vi "Main Page.vi"(8 "error in (no error)":errorcluster, 11 "Node Ptr":T4 format="%.0x") -> (0 "error out":errorcluster)   [LabVIEW 2024, in "Diagnostics Addon System Explorer.lvlib"]
uses:
  Diagnostics Addon System Explorer.lvlib
  <vilib>/NI VeriStand/Custom Device API/Custom Device API.lvlib
  Types/FG.Action.ctl
  Addon Shared/Types/986x.ctl
  Addon Shared/Diagnostics Addon Shared.lvlib
  <vilib>/NI/NI VeriStand Hardware Resource Discovery/NIVS Hardware Discovery.lvlib
  <vilib>/NI/NI VeriStand Hardware Resource Discovery/_Types/Filter Type.ctl
  Addon Shared/SubVIs/Constants.vi
  <vilib>/NI VeriStand/Custom Device API/Custom Device Item Ref.ctl
  Addon Shared/Types/Protocol.ctl
  Addon Shared/Types/Transport.ctl
panel:
  in  "Tab Control":T1(tab)
  in  "Dynamic Port":bool=TRUE
  in  "DoIP Version":u16(ring)=2 items=["2010"=1, "2012"=2]
  in  "Address":string
  in  "FD ISO Mode":u32(ring) items=["ISO", "Non ISO", "ISO Legacy"]
  in  "CAN Browse":bool
  out "Version":string
  in  "Termination":enum16{"Off", "On"}(ring)
  in  "Name":string
  in  "Description":string
  out "Diagnostic Protocol":T2
  in  "Port":string
  in  "Baud Rate":u64=250000
  in  "Enable Stream":bool
  in  "FD Baud Rate":u64=250000
  in  "Max DLC":u16
  in  "IO Mode":u32(ring) items=["CAN 2.0", "CAN FD", "CAN FD+BRS"]
  in  "Transport Protocol":T3
  in  "Source Address":u16=3584 format="%.0x"
  in  "Timeout":u32 caption="Comm Timeout (ms)"
  in  "Fill Byte":u8=255 format="%.0x"
  in  "Fill Frame":bool
  in  "VW TP Channel ID":u32 format="%.0x"
  in  "Receive UUDT ID":u32 format="%.0x"
  in  "Receive Extension":u8 format="%.0x"
  in  "Receive ID":u32 format="%.0x"
  in  "Transmit Extension":u8 format="%.0x"
  in  "Transmit ID":u32 format="%.0x"
  in  "NAD":u8
  in  "LIN Cluster":refnum<k21>
  in  "RIO Browse":bool
  in  "RIO Device":string
  in  "Enable Bitfile":bool
  in  "Bitfile Path":path
  in  "Header":cluster{"Section Name":string}={"Section Name"="Addon Settings"}
  in  "SHDocVw.IWebBrowser":refnum<k7>(container)
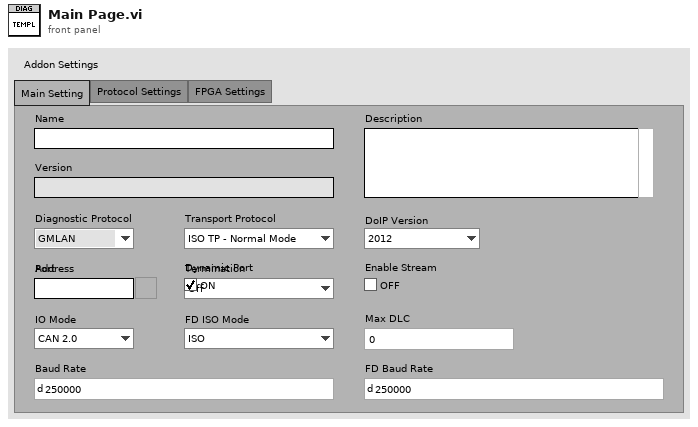
[diagram p1: front panel]
types:
  T1 = enum32{"Main Setting", "Protocol Settings", "FPGA Settings"}
  T2 = typedef "Diagnostics Addon Shared.lvlib/Protocol.ctl" = enum16{"GMLAN", "KWP-2000", "UDS", "User-Defined"}
  T3 = typedef "Diagnostics Addon Shared.lvlib/Transport.ctl" = enum16{"ISO TP - Normal Mode", "ISO TP - Mixed Mode", "VW TP 2.0", "Diagnostics on IP", "ISO TP LIN"}
  T4 = typedef "Custom Device API.lvlib/Custom Device Item Ref.ctl" = u64
  T5 = typedef "Diagnostics Addon System Explorer.lvlib/FG.Action.ctl" = enum16{"Get", "Set"}
  T6 = typedef "Custom Device API.lvlib/Custom Device Item Info.ctl" = cluster{"Name":string, "Is Channel":bool, "GUID":string, "Is Waveform":bool}
  T7 = typedef "Diagnostics Addon Shared.lvlib/986x.ctl" = cluster{"Enable":bool, "RIO Device":string, "Bitfile":path}
  T8 = typedef "Diagnostics Addon Shared.lvlib/CAN.ctl" = cluster{"Interface":T9, "Baud Rate":u64, "Diagnostic Protocol":T2, "Transport Protocol":T3, "Transmit ID":u32, "Receive ID":u32, "Transmit Extension":u8, "Receive Extension":u8, "Receive UUDT ID":u32, "Enable Stream":bool, "VW TP Channel ID":u32, "Fill Frame":bool, "Fill Byte":u8, "Termination":bool, "LIN Cluster":refnum<k21>, "NAD":u8, "IO Mode":u32, "Max DLC":u16, "FD Baud Rate":u64, "Timeout":u32, "FD ISO Mode":u32, "DoIP Address":string, "DoIP Source Address":u16, "DoIP Dynamic Port":bool, "DoIP Version":u16}
  T9 = typedef "Diagnostics Addon Shared.lvlib/CAN.Interface.ctl" = string
  T10 = typedef "NIVS Hardware Discovery.lvlib/Filter Type.ctl" = enum16{"Device Category", "Product Name", "Ethernet", "XNET", "VISA", "FPGA", "EtherCAT Master", "DAQmx", "GPIB", "Serial"}
  T11 = typedef "Custom Device API.lvlib/Custom Device Commands.ctl" = enum16{"Default", "Item renamed", "Shutdown", "Dynamic button pressed"}
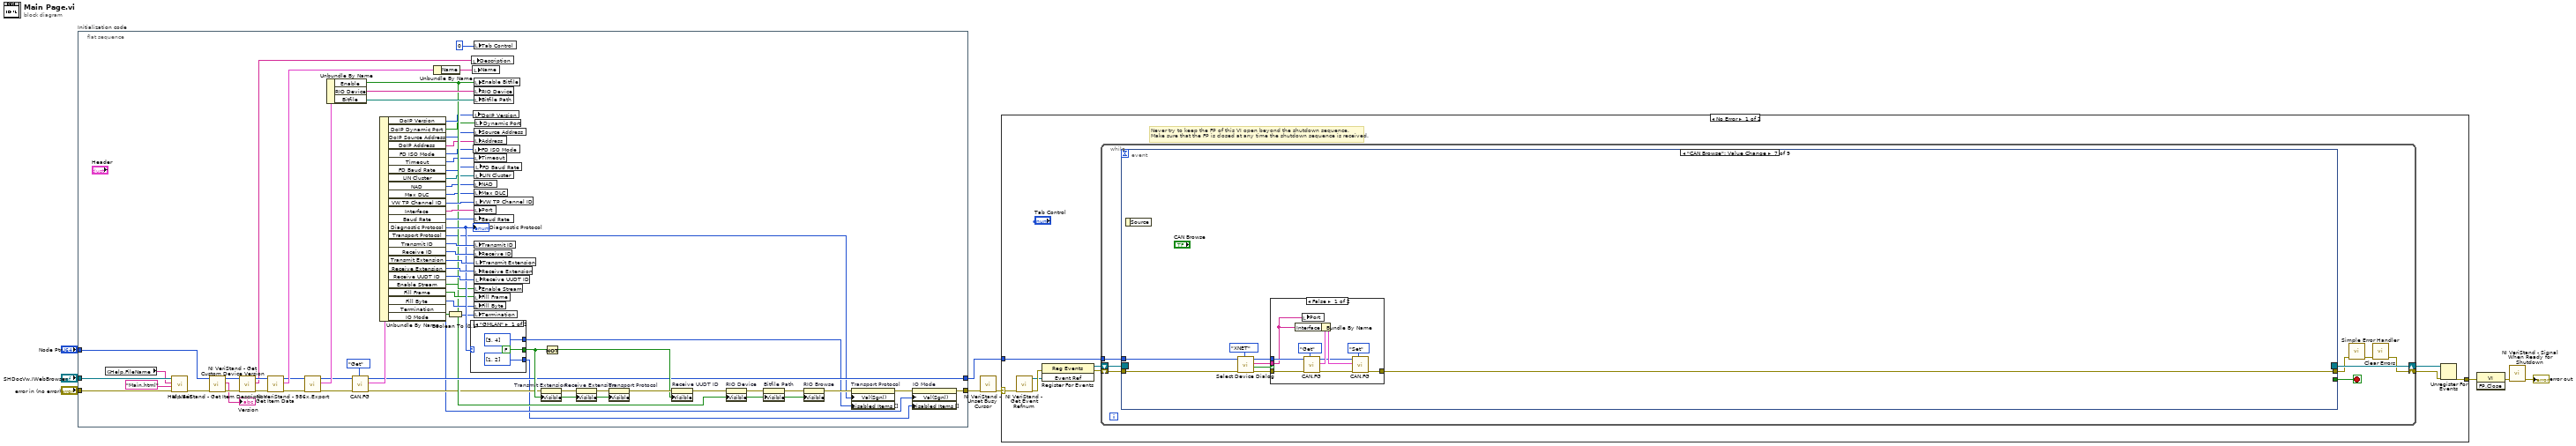
[diagram p0: block diagram]
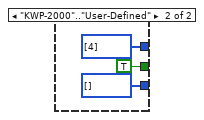
[diagram p2: hidden frame]
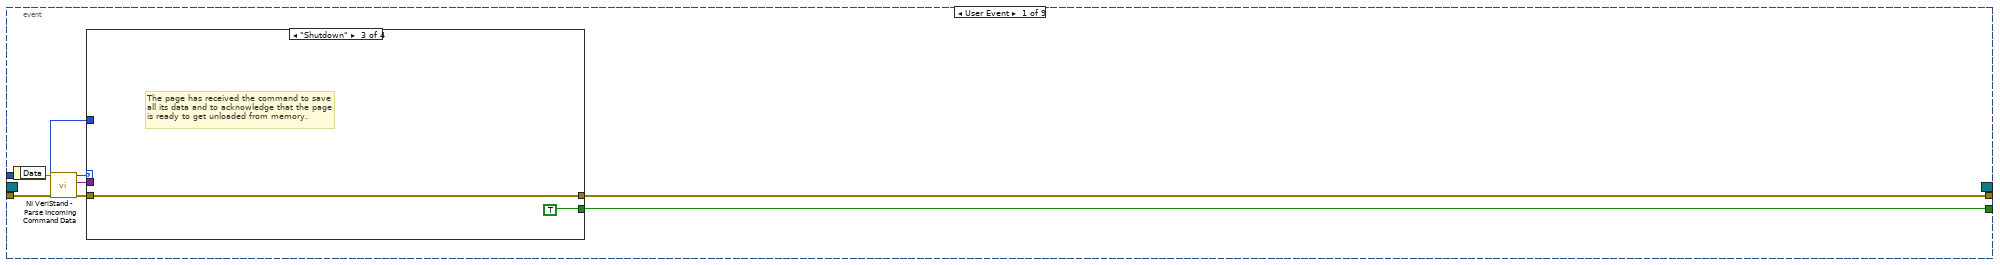
[diagram p3: hidden frame]
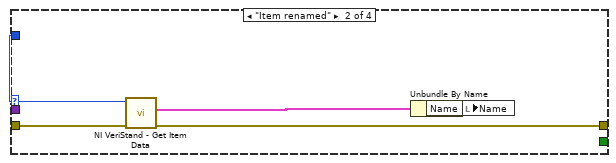
[diagram p5: hidden frame]
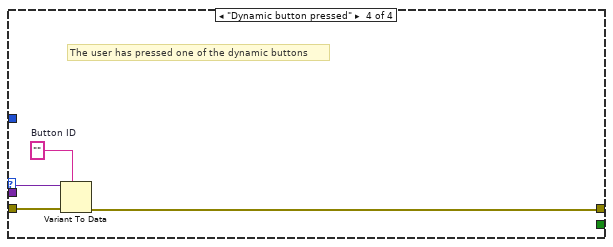
[diagram p6: hidden frame]
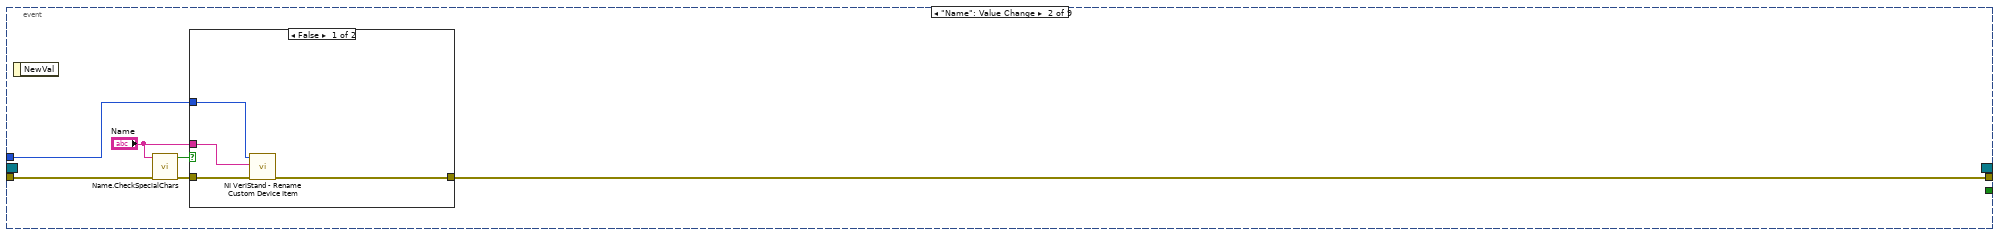
[diagram p7: hidden frame]
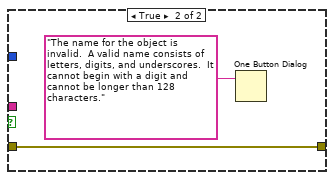
[diagram p8: hidden frame]
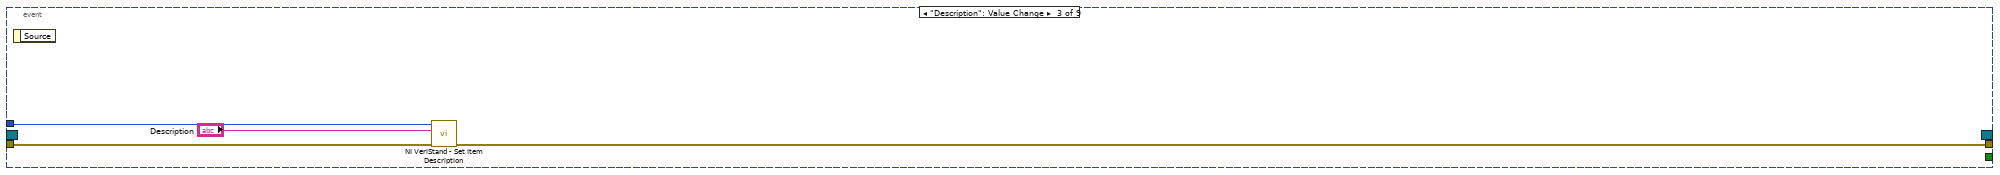
[diagram p9: hidden frame]
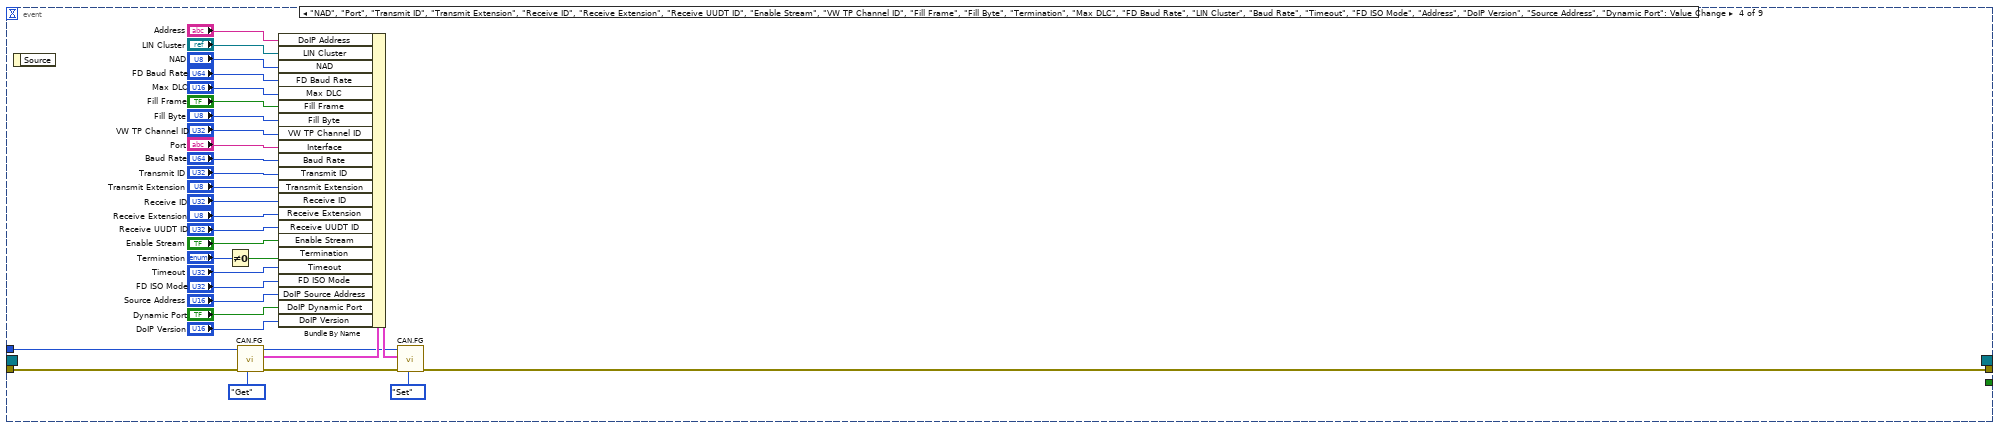
[diagram p10: hidden frame]
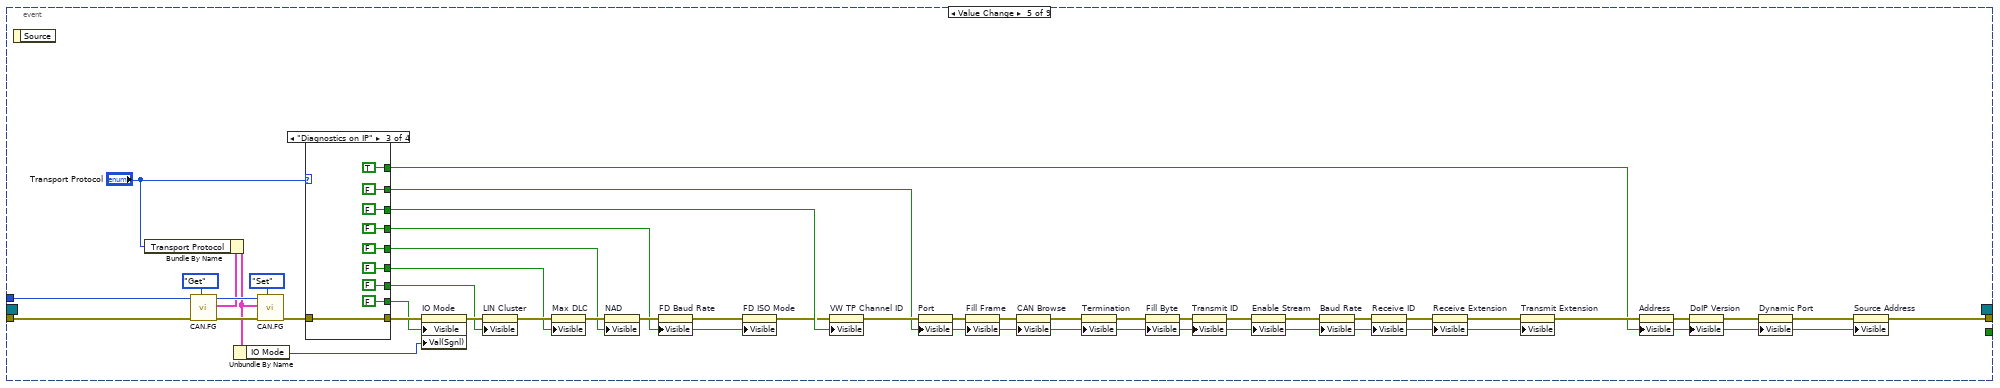
[diagram p11: hidden frame]
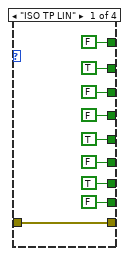
[diagram p12: hidden frame]
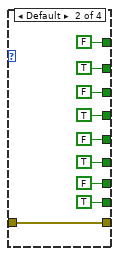
[diagram p13: hidden frame]
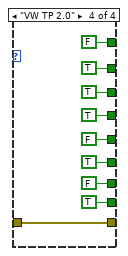
[diagram p14: hidden frame]
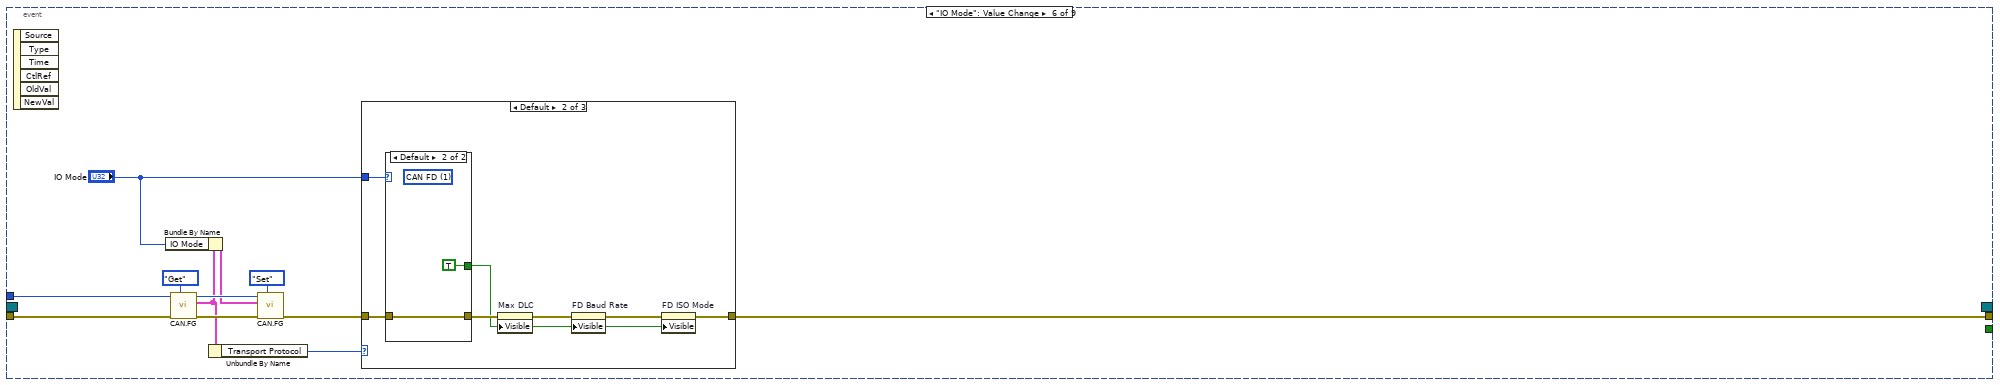
[diagram p15: hidden frame]
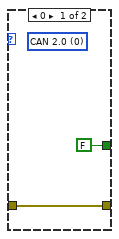
[diagram p17: hidden frame]
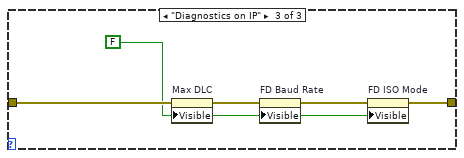
[diagram p18: hidden frame]
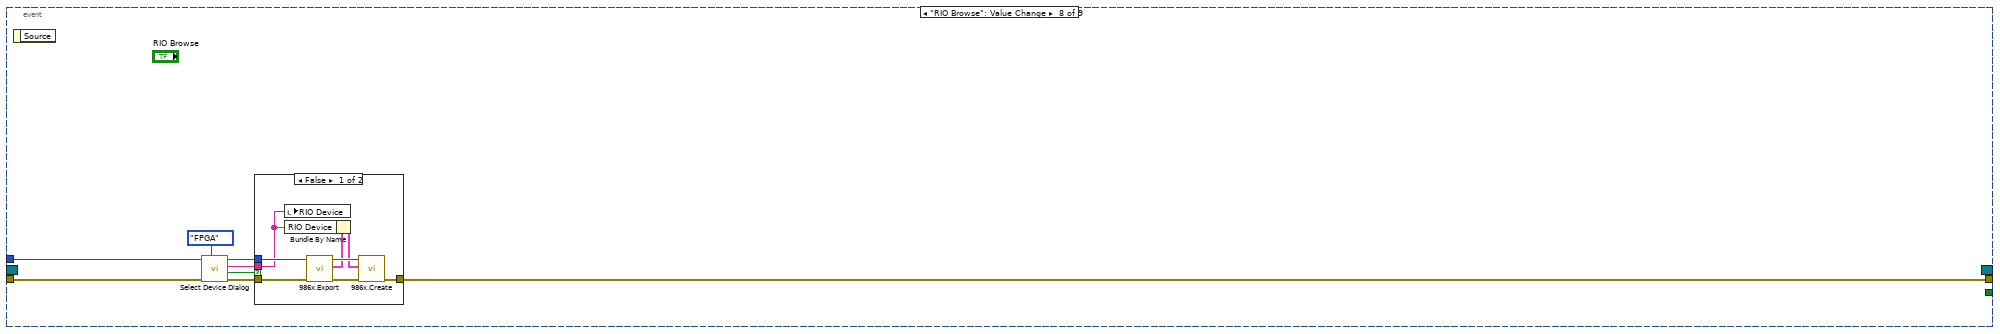
[diagram p20: hidden frame]
diagram:
  n1 = flat-sequence "Initialization code" {
    tunnel: "error in (no error)" -> [w70]
    tunnel: "Node Ptr" -> [w37]
    tunnel: [w19] -> w5
    tunnel: [w39] -> w2
    tunnel: "SHDocVw.IWebBrowser" -> [w69]
    frame #0 {
      n2 = global read "Constants.vi" "Help.FileName"() -> (w21:string)
      n3 = call "Help.Set.vi"("error in (no error)"=w70, "HTML File"="Main.html", "Main CHM File"=w21, "SHDocVw.IWebBrowser2"=w69) -> ("error out"=w38:errorcluster)  [unwired: 7 in]
      n4 = call <vilib>:"NI VeriStand - Get Custom Device Version.vi"("error in (no error)"=w38, "Device Ref in"=w37) -> ("error out"=w35:errorcluster, "Value"=→"Version":string, "Device Ref out"=w36:T4)  [unwired: 7 in]
      n5 = call <vilib>:"NI VeriStand - Get Item Description.vi"("error in (no error)"=w35, "Item Ref in"=w36) -> ("error out"=w73:errorcluster, "Description"=w74:string, "Item Ref out"=w75:T4)  [unwired: 7 out]
      n6 = call <vilib>:"NI VeriStand - Get Item Data.vi"("error in (no error)"=w73, "Item Ref in"=w75) -> ("error out"=w45:errorcluster, "Item Info"=w72:T6, "Item Ref out"=w44:T4)  [unwired: 7 out]
      n7 = call "986x.Export.vi"("error in (no error)"=w45, "Device Item Ref in"=w44) -> ("error out"=w43:errorcluster, "986x Support"=w46:T7, "Item Ref out"=w42:T4)  [unwired: 7 in]
      n8 = Unbundle By Name(w46) -> ("Enable"=w30:bool, "RIO Device"=w40:string, "Bitfile"=w41:path)
      n9 = call "CAN.FG.vi"("Action"=FG.Action."Get", "error in (no error)"=w43, "Device Item Ref in"=w42) -> ("error out"=w23:errorcluster, "Diagnostics Basic Configuration"=w67:T8, "Device Item Ref out"=w39:T4)  [unwired: 6 in]
      n10 = Unbundle By Name(w67) -> ("DoIP Version"=w12:u16, "DoIP Dynamic Port"=w11:bool, "DoIP Source Address"=w10:u16, "DoIP Address"=w13:string, "FD ISO Mode"=w15:u32, "Timeout"=w22:u32, "FD Baud Rate"=w29:u64, "LIN Cluster"=w25:refnum<k21>, "NAD"=w28:u8, "Max DLC"=w27:u16, "VW TP Channel ID"=w53:u32, "Interface"=w66:T9, "Baud Rate"=w65:u64, "Diagnostic Protocol"=w59:T2, "Transport Protocol"=w24:T3, "Transmit ID"=w64:u32, "Receive ID"=w63:u32, "Transmit Extension"=w62:u8, "Receive Extension"=w60:u8, "Receive UUDT ID"=w61:u32, "Enable Stream"=w54:bool, "Fill Frame"=w48:bool, "Fill Byte"=w49:u8, "Termination"=w47:bool, "IO Mode"=w18:u32)
      "Diagnostic Protocol" <- w59
      n11 = Unbundle By Name(w72) -> ("Name"=w71:string)
      n12 = Boolean To (0,1)(Boolean=w47) -> (0, 1=w16:i16)
      n13 = case shown="\"GMLAN\"" w59 {
        tunnel: [FALSE TRUE] -> w51
        tunnel: [i32[] [1, 2] ("Disabled Items []") i32[] [] ("Disabled Items []")] -> w17
        tunnel: [i32[] [3, 4] ("Disabled Items []") i32[] [4] ("Disabled Items []")] -> w14
        frame "GMLAN" {
        }
        frame "KWP-2000".."User-Defined" {
        }
      }
      n14 = local write "Description"(w74) -> ()
      n15 = local write "Name"(w71) -> ()
      n16 = local write "DoIP Version"(w12) -> ()
      n17 = local write "FD ISO Mode"(w15) -> ()
      n18 = local write "Tab Control"(0) -> ()
      n19 = local write "Enable Bitfile"(w30) -> ()
      n20 = local write "RIO Device"(w40) -> ()
      n21 = local write "Bitfile Path"(w41) -> ()
      n22 = local write "Source Address"(w10) -> ()
      n23 = local write "Address"(w13) -> ()
      n24 = local write "Timeout"(w22) -> ()
      n25 = local write "NAD"(w28) -> ()
      n26 = local write "Max DLC"(w27) -> ()
      n27 = local write "Port"(w66) -> ()
      n28 = local write "Baud Rate"(w65) -> ()
      n29 = local write "Transmit ID"(w64) -> ()
      n30 = local write "Receive ID"(w63) -> ()
      n31 = local write "Receive Extension"(w60) -> ()
      n32 = local write "Enable Stream"(w54) -> ()
      n33 = local write "Fill Frame"(w48) -> ()
      n34 = local write "Fill Byte"(w49) -> ()
      n35 = local write "Termination"(w16) -> ()
      n36 = local write "FD Baud Rate"(w29) -> ()
      n37 = local write "LIN Cluster"(w25) -> ()
      n38 = local write "VW TP Channel ID"(w53) -> ()
      n39 = local write "Transmit Extension"(w62) -> ()
      n40 = local write "Receive UUDT ID"(w61) -> ()
      n41 = local write "Dynamic Port"(w11) -> ()
      n42 = property on="Transmit Extension" class="DigNum (strict)"(error in=w23, "Visible"=w51) -> (error out=w58:errorcluster)  [unwired: 1 in, 1 out]
      n43 = Not(x=w51) -> (.not. x?=w55:bool)
      n44 = property on="Receive Extension" class="DigNum (strict)"(error in=w58, "Visible"=w51) -> (error out=w57:errorcluster)  [unwired: 1 in, 1 out]
      n45 = property on="Transport Protocol" class="Enum (strict)"(error in=w57, "Visible"=w51) -> (error out=w56:errorcluster)  [unwired: 1 in, 1 out]
      n46 = property on="Receive UUDT ID" class="DigNum (strict)"(error in=w56, "Visible"=w55) -> (error out=w31:errorcluster)  [unwired: 1 in, 1 out]
      n47 = property on="RIO Device" class="Str"(error in=w31, "Visible"=w30) -> (error out=w33:errorcluster)  [unwired: 1 in, 1 out]
      n48 = property on="Bitfile Path" class="Path"(error in=w33, "Visible"=w30) -> (error out=w32:errorcluster)  [unwired: 1 in, 1 out]
      n49 = property on="RIO Browse" class="Bool"(error in=w32, "Visible"=w30) -> (error out=w26:errorcluster)  [unwired: 1 in, 1 out]
      n50 = property on="Transport Protocol" class="Enum (strict)"(error in=w26, "Val(Sgnl)"=w24, "Disabled Items []"=w14) -> (error out=w20:errorcluster)  [unwired: 1 in, 1 out]
      n51 = property on="IO Mode" class="Ring (strict)"(error in=w20, "Val(Sgnl)"=w18, "Disabled Items []"=w17) -> (error out=w19:errorcluster)  [unwired: 1 in, 1 out]
    }
  }
  n52 = call <vilib>:"NI VeriStand - Unset Busy Cursor.vi"("error in (no error)"=w5) -> ("error out"=w4:errorcluster)  [unwired: 10 out]
  n53 = case shown="No Error" w4 {
    selector: w4 -> [w82 w323]
    tunnel: [w87 w321] -> w9
    tunnel: w2 -> [w83 _]
    frame No Error {
      # "Never try to keep the FP of this VI open beyond the shutdown sequence.\nMake sure that the FP is closed at any time the shutdown sequence is received."
      n54 = call <vilib>:"NI VeriStand - Get Event Refnum.vi"("error in (no error)"=w82) -> ("error out"=w90:errorcluster, "Event Ref"=w86:refnum<user-event>)  [unwired: 9 out]
      n55 = register-events(error in=w90, w86) -> (reference out=w84:refnum<event-registration>, error out=w85:errorcluster)  [unwired: 1 in]
      n56 = while {
        tunnel: w83 -> [w94]
        shift-right: [w91] -> w88
        shift-left: w85 -> [w97]
        shift-right: [w98] -> w89
        shift-left: w84 -> [w96]
        stop <- w95 stop-if-true
        n57 = event shown="[6] \"CAN Browse\": Value Change" {
          selector: w96 -> [_ _ _ _ _ _ _ _ _]
          dyn-events: [_ _ _ _ _ _ _ _ _] -> w98
          timeout: _ -> [_ _ _ _ _ _ _ _ _]
          tunnel: w97 -> [w106 w121 w133 w166 w208 w256 w280 w298 w315]
          tunnel: [w102 _ _ _ _ _ _ _ _] -> w95
          tunnel: [w101 w124 w132 w150 w170 w248 w281 w300 w317] -> w93
          tunnel: w94 -> [w100 w123 w134 w165 w207 w255 w279 w296 w316]
          event User Event {
            n58 = event-data() -> ("Data"=w105:string)  [unwired: 1 out]
            n59 = call <vilib>:"NI VeriStand - Parse Incoming Command Data.vi"("error in (no error)"=w106, "Incoming data"=w105) -> ("error out"=w104:errorcluster, "Outgoing data"=w99:variant, "Action"=w103:T11)  [unwired: 7 out]
            n60 = case shown="\"Shutdown\"" w103 {
              tunnel: w104 -> [w107 w112 w113 w118]
              tunnel: [_ _ TRUE _] -> w102
              tunnel: [w107 w109 w113 w115] -> w101
              tunnel: w100 -> [_ w111 _ _]
              tunnel: w99 -> [_ _ _ w117]
              frame "Default", Default {
              }
              frame "Item renamed" {
                n61 = call <vilib>:"NI VeriStand - Get Item Data.vi"("error in (no error)"=w112, "Item Ref in"=w111) -> ("error out"=w109:errorcluster, "Item Info"=w110:T6)  [unwired: 8 out]
                n62 = Unbundle By Name(w110) -> ("Name"=w108:string)
                n63 = local write "Name"(w108) -> ()
              }
              frame "Shutdown" {
                # "The page has received the command to save all its data and to acknowledge that the page is ready to get unloaded from memory."
              }
              frame "Dynamic button pressed" {
                w116 = ""  # Button ID
                # "The user has pressed one of the dynamic buttons"
                n64 = Variant To Data(error in=w118, type=w116, Variant=w117) -> (error out=w115:errorcluster)  [unwired: 1 out]
              }
            }
          }
          event "Name": Value Change {
            n65 = event-data() -> ()  [unwired: 2 out]
            n66 = call "Name.CheckSpecialChars.vi"("error in"=w121, "Signal Name"="Name") -> ("error out"=w120:errorcluster, "Special Character?"=w119:bool)  [unwired: 8 in]
            n67 = case shown="False" w119 {
              tunnel: [w128 w130] -> w124
              tunnel: w123 -> [w127 _]
              tunnel: "Name" -> [w126 _]
              tunnel: w120 -> [w125 w130]
              frame False {
                n68 = call <vilib>:"NI VeriStand - Rename Custom Device Item.vi"("error in (no error)"=w125, "New Name"=w126, "Item Ref in"=w127) -> ("error out"=w128:errorcluster)  [unwired: 1 in, 7 out]
              }
              frame True {
                n69 = One Button Dialog(message="The name for the object is invalid.  A valid name consists of letters, digits, and underscores.  It cannot begin with a digit and cannot be longer than 128 characters.") -> ()  [unwired: 1 in, 1 out]
              }
            }
          }
          event "Description": Value Change {
            n70 = event-data() -> ()  [unwired: 2 out]
            n71 = call <vilib>:"NI VeriStand - Set Item Description.vi"("error in (no error)"=w133, "Description"="Description", "Item Ref in"=w134) -> ("error out"=w132:errorcluster)  [unwired: 8 out]
          }
          event "NAD", "Port", "Transmit ID", "Transmit Extension", "Receive ID", "Receive Extension", "Receive UUDT ID", "Enable Stream", "VW TP Channel ID", "Fill Frame", "Fill Byte", "Termination", "Max DLC", "FD Baud Rate", "LIN Cluster", "Baud Rate", "Timeout", "FD ISO Mode", "Address", "DoIP Version", "Source Address", "Dynamic Port": Value Change {
            n72 = event-data() -> ()  [unwired: 2 out]
            n73 = Not Equal To 0?(x="Termination") -> (x != 0?=w140:bool)
            n74 = call "CAN.FG.vi"("Action"=FG.Action."Get", "error in (no error)"=w166, "Device Item Ref in"=w165) -> ("error out"=w152:errorcluster, "Diagnostics Basic Configuration"=w164:T8, "Device Item Ref out"=w151:T4)  [unwired: 6 in]
            n75 = Bundle By Name(cluster=w164, "DoIP Address"="Address", "LIN Cluster"="LIN Cluster", "NAD"="NAD", "FD Baud Rate"="FD Baud Rate", "Max DLC"="Max DLC", "Fill Frame"="Fill Frame", "Fill Byte"="Fill Byte", "VW TP Channel ID"="VW TP Channel ID", "Interface"="Port", "Baud Rate"="Baud Rate", "Transmit ID"="Transmit ID", "Transmit Extension"="Transmit Extension", "Receive ID"="Receive ID", "Receive Extension"="Receive Extension", "Receive UUDT ID"="Receive UUDT ID", "Enable Stream"="Enable Stream", "Termination"=w140, "Timeout"="Timeout", "FD ISO Mode"="FD ISO Mode", "DoIP Source Address"="Source Address", "DoIP Dynamic Port"="Dynamic Port", "DoIP Version"="DoIP Version") -> (w153:T8)
            n76 = call "CAN.FG.vi"("Action"=FG.Action."Set", "error in (no error)"=w152, "Diagnostics Basic Configuration"=w153, "Device Item Ref in"=w151) -> ("error out"=w150:errorcluster)  [unwired: 5 in, 2 out]
          }
          event Value Change {
            n77 = event-data() -> ()  [unwired: 2 out]
            n78 = call "CAN.FG.vi"("Action"=FG.Action."Get", "error in (no error)"=w208, "Device Item Ref in"=w207) -> ("error out"=w205:errorcluster, "Diagnostics Basic Configuration"=w202:T8, "Device Item Ref out"=w204:T4)  [unwired: 6 in]
            n79 = Bundle By Name(cluster=w202, "Transport Protocol"="Transport Protocol") -> (w190:T8)
            n80 = Unbundle By Name(w190) -> ("IO Mode"=w172:u32)
            n81 = call "CAN.FG.vi"("Action"=FG.Action."Set", "error in (no error)"=w205, "Diagnostics Basic Configuration"=w190, "Device Item Ref in"=w204) -> ("error out"=w200:errorcluster)  [unwired: 5 in, 2 out]
            n82 = case shown="\"Diagnostics on IP\"" "Transport Protocol" {
              tunnel: w200 -> [w217 w226 w235 w244]
              tunnel: [w217 w226 w235 w244] -> w195
              tunnel: [FALSE ("Visible") TRUE ("Visible") FALSE ("Visible") TRUE ("Visible")] -> w194
              tunnel: [TRUE ("Visible") FALSE ("Visible") FALSE ("Visible") FALSE ("Visible")] -> w193
              tunnel: [FALSE ("Visible") TRUE ("Visible") FALSE ("Visible") TRUE ("Visible")] -> w192
              tunnel: [TRUE ("Visible") FALSE ("Visible") FALSE ("Visible") FALSE ("Visible")] -> w191
              tunnel: [FALSE ("Visible") TRUE ("Visible") FALSE ("Visible") TRUE ("Visible")] -> w186
              tunnel: [FALSE ("Visible") FALSE ("Visible") FALSE ("Visible") TRUE ("Visible")] -> w189
              tunnel: [TRUE TRUE FALSE TRUE] -> w174
              tunnel: [FALSE ("Visible") FALSE ("Visible") TRUE ("Visible") FALSE ("Visible")] -> w167
              frame "ISO TP LIN" {
              }
              frame Default {
              }
              frame "Diagnostics on IP" {
              }
              frame "VW TP 2.0" {
              }
            }
            n83 = property on="IO Mode" class="Ring (strict)"(error in=w195, "Visible"=w194, "Val(Sgnl)"=w172) -> (error out=w197:errorcluster)  [unwired: 1 in, 1 out]
            n84 = property on="LIN Cluster" class="XNET (strict)"(error in=w197, "Visible"=w193) -> (error out=w196:errorcluster)  [unwired: 1 in, 1 out]
            n85 = property on="Max DLC" class="DigNum (strict)"(error in=w196, "Visible"=w192) -> (error out=w198:errorcluster)  [unwired: 1 in, 1 out]
            n86 = property on="NAD" class="DigNum (strict)"(error in=w198, "Visible"=w191) -> (error out=w199:errorcluster)  [unwired: 1 in, 1 out]
            n87 = property on="FD Baud Rate" class="DigNum (strict)"(error in=w199, "Visible"=w186) -> (error out=w188:errorcluster)  [unwired: 1 in, 1 out]
            n88 = property on="FD ISO Mode" class="Ring (strict)"(error in=w188, "Visible"=w186) -> (error out=w187:errorcluster)  [unwired: 1 in, 1 out]
            n89 = property on="VW TP Channel ID" class="DigNum (strict)"(error in=w187, "Visible"=w189) -> (error out=w177:errorcluster)  [unwired: 1 in, 1 out]
            n90 = property on="Port" class="Str"(error in=w177, "Visible"=w174) -> (error out=w185:errorcluster)  [unwired: 1 in, 1 out]
            n91 = property on="Fill Frame" class="Bool (strict)"(error in=w185, "Visible"=w174) -> (error out=w184:errorcluster)  [unwired: 1 in, 1 out]
            n92 = property on="CAN Browse" class="Bool"(error in=w184, "Visible"=w174) -> (error out=w183:errorcluster)  [unwired: 1 in, 1 out]
            n93 = property on="Termination" class="Enum (strict)"(error in=w183, "Visible"=w174) -> (error out=w182:errorcluster)  [unwired: 1 in, 1 out]
            n94 = property on="Fill Byte" class="DigNum (strict)"(error in=w182, "Visible"=w174) -> (error out=w181:errorcluster)  [unwired: 1 in, 1 out]
            n95 = property on="Transmit ID" class="DigNum (strict)"(error in=w181, "Visible"=w174) -> (error out=w180:errorcluster)  [unwired: 1 in, 1 out]
            n96 = property on="Enable Stream" class="Bool (strict)"(error in=w180, "Visible"=w174) -> (error out=w179:errorcluster)  [unwired: 1 in, 1 out]
            n97 = property on="Baud Rate" class="DigNum (strict)"(error in=w179, "Visible"=w174) -> (error out=w178:errorcluster)  [unwired: 1 in, 1 out]
            n98 = property on="Receive ID" class="DigNum (strict)"(error in=w178, "Visible"=w174) -> (error out=w175:errorcluster)  [unwired: 1 in, 1 out]
            n99 = property on="Receive Extension" class="DigNum (strict)"(error in=w175, "Visible"=w174) -> (error out=w176:errorcluster)  [unwired: 1 in, 1 out]
            n100 = property on="Transmit Extension" class="DigNum (strict)"(error in=w176, "Visible"=w174) -> (error out=w173:errorcluster)  [unwired: 1 in, 1 out]
            n101 = property on="Address" class="Str"(error in=w173, "Visible"=w167) -> (error out=w171:errorcluster)  [unwired: 1 in, 1 out]
            n102 = property on="DoIP Version" class="Ring (strict)"(error in=w171, "Visible"=w167) -> (error out=w168:errorcluster)  [unwired: 1 in, 1 out]
            n103 = property on="Dynamic Port" class="Bool (strict)"(error in=w168, "Visible"=w167) -> (error out=w169:errorcluster)  [unwired: 1 in, 1 out]
            n104 = property on="Source Address" class="DigNum (strict)"(error in=w169, "Visible"=w167) -> (error out=w170:errorcluster)  [unwired: 1 in, 1 out]
          }
          event "IO Mode": Value Change {
            n105 = event-data() -> ()  [unwired: 7 out]
            n106 = call "CAN.FG.vi"("Action"=FG.Action."Get", "error in (no error)"=w256, "Device Item Ref in"=w255) -> ("error out"=w253:errorcluster, "Diagnostics Basic Configuration"=w246:T8, "Device Item Ref out"=w252:T4)  [unwired: 6 in]
            n107 = Bundle By Name(cluster=w246, "IO Mode"="IO Mode") -> (w250:T8)
            n108 = Unbundle By Name(w246) -> ("Transport Protocol"=w245:T3)
            n109 = call "CAN.FG.vi"("Action"=FG.Action."Set", "error in (no error)"=w253, "Diagnostics Basic Configuration"=w250, "Device Item Ref in"=w252) -> ("error out"=w249:errorcluster)  [unwired: 5 in, 2 out]
            n110 = case shown="Default" w245 {
              tunnel: w249 -> [w257 w264 w273]
              tunnel: [w257 w259 w270] -> w248
              tunnel: "IO Mode" -> [_ w263 _]
              frame "ISO TP LIN" {
              }
              frame Default {
                n111 = case shown="Default" w263 {
                  tunnel: w264 -> [w266 w268]
                  tunnel: [w266 w268] -> w262
                  tunnel: [FALSE ("Visible") TRUE ("Visible")] -> w258
                  frame 0 {
                    (unwired) u32 0 items=["CAN 2.0", "CAN FD", "CAN FD+BRS"] ("IO Mode")
                  }
                  frame Default {
                    (unwired) u32 1 items=["CAN 2.0", "CAN FD", "CAN FD+BRS"] ("IO Mode")
                  }
                }
                n112 = property on="Max DLC" class="DigNum (strict)"(error in=w262, "Visible"=w258) -> (error out=w261:errorcluster)  [unwired: 1 in, 1 out]
                n113 = property on="FD Baud Rate" class="DigNum (strict)"(error in=w261, "Visible"=w258) -> (error out=w260:errorcluster)  [unwired: 1 in, 1 out]
                n114 = property on="FD ISO Mode" class="Ring (strict)"(error in=w260, "Visible"=w258) -> (error out=w259:errorcluster)  [unwired: 1 in, 1 out]
              }
              frame "Diagnostics on IP" {
                w269 = FALSE ("Visible")
                n115 = property on="Max DLC" class="DigNum (strict)"(error in=w273, "Visible"=w269) -> (error out=w272:errorcluster)  [unwired: 1 in, 1 out]
                n116 = property on="FD Baud Rate" class="DigNum (strict)"(error in=w272, "Visible"=w269) -> (error out=w271:errorcluster)  [unwired: 1 in, 1 out]
                n117 = property on="FD ISO Mode" class="Ring (strict)"(error in=w271, "Visible"=w269) -> (error out=w270:errorcluster)  [unwired: 1 in, 1 out]
              }
            }
          }
          event "CAN Browse": Value Change {
            n118 = event-data() -> ()  [unwired: 2 out]
            n119 = call <vilib>:"Select Device Dialog.vi"("Filter Type"=Filter_Type."XNET", "error in (no error)"=w280, "Item Ref in"=w279) -> ("error out"=w277:errorcluster, "Cancelled?"=w274:bool, "Selected Alias"=w275:string, "Item Ref out"=w278:T4)  [unwired: 5 in]
            n120 = case shown="False" w274 {
              tunnel: [w286 w292] -> w281
              tunnel: w278 -> [w284 _]
              tunnel: w277 -> [w283 w292]
              tunnel: w275 -> [w282 _]
              frame False {
                n121 = local write "Port"(w282) -> ()
                n122 = call "CAN.FG.vi"("Action"=FG.Action."Get", "error in (no error)"=w283, "Device Item Ref in"=w284) -> ("error out"=w288:errorcluster, "Diagnostics Basic Configuration"=w291:T8, "Device Item Ref out"=w287:T4)  [unwired: 6 in]
                n123 = Bundle By Name(cluster=w291, "Interface"=w282) -> (w289:T8)
                n124 = call "CAN.FG.vi"("Action"=FG.Action."Set", "error in (no error)"=w288, "Diagnostics Basic Configuration"=w289, "Device Item Ref in"=w287) -> ("error out"=w286:errorcluster)  [unwired: 5 in, 2 out]
              }
              frame True {
              }
            }
          }
          event "RIO Browse": Value Change {
            n125 = event-data() -> ()  [unwired: 2 out]
            n126 = call <vilib>:"Select Device Dialog.vi"("Filter Type"=Filter_Type."FPGA", "error in (no error)"=w298, "Item Ref in"=w296) -> ("error out"=w297:errorcluster, "Cancelled?"=w293:bool, "Selected Alias"=w294:string, "Item Ref out"=w295:T4)  [unwired: 5 in]
            n127 = case shown="False" w293 {
              tunnel: [w308 w309] -> w300
              tunnel: w297 -> [w303 w309]
              tunnel: w295 -> [w302 _]
              tunnel: w294 -> [w301 _]
              frame False {
                n128 = local write "RIO Device"(w301) -> ()
                n129 = call "986x.Export.vi"("error in (no error)"=w303, "Device Item Ref in"=w302) -> ("error out"=w307:errorcluster, "986x Support"=w305:T7, "Item Ref out"=w306:T4)  [unwired: 7 in]
                n130 = Bundle By Name(cluster=w305, "RIO Device"=w301) -> (w304:T7)
                n131 = call "986x.Create.vi"("error in (no error)"=w307, "986x Support"=w304, "Device Item Ref in"=w306) -> ("error out"=w308:errorcluster)  [unwired: 7 in, 1 out]
              }
              frame True {
              }
            }
          }
          event "Enable Bitfile", "Bitfile Path", "RIO Device": Value Change {
            n132 = event-data() -> ()  [unwired: 2 out]
            n133 = property on="RIO Device" class="Str"(error in=w315, "Visible"="Enable Bitfile") -> (error out=w314:errorcluster)  [unwired: 1 in, 1 out]
            n134 = Bundle By Name(cluster=T7 {"Enable"=FALSE, "RIO Device"="", "Bitfile"=path ""} ("986x Support"), "RIO Device"="RIO Device", "Bitfile"="Bitfile Path", "Enable"="Enable Bitfile") -> (w318:T7)
            n135 = property on="Bitfile Path" class="Path"(error in=w314, "Visible"="Enable Bitfile") -> (error out=w312:errorcluster)  [unwired: 1 in, 1 out]
            n136 = property on="RIO Browse" class="Bool"(error in=w312, "Visible"="Enable Bitfile") -> (error out=w311:errorcluster)  [unwired: 1 in, 1 out]
            n137 = call "986x.Create.vi"("error in (no error)"=w311, "986x Support"=w318, "Device Item Ref in"=w316) -> ("error out"=w317:errorcluster)  [unwired: 7 in, 1 out]
          }
        }
        n138 = call <vilib>:"Simple Error Handler.vi"("error in (no error)"=w93) -> ("error out"=w92:errorcluster)  [unwired: 1 in, 7 out]
        n139 = call <vilib>:"Clear Errors.vi"("error in (no error)"=w92) -> ("error out"=w91:errorcluster)  [unwired: 1 in, 5 out]
      }
      n140 = Unregister For Events(event registration refnum=w89, error in=w88) -> (error out=w87:errorcluster)
    }
    frame Error {
      n141 = call <vilib>:"Simple Error Handler.vi"("error in (no error)"=w323) -> ("error out"=w322:errorcluster)  [unwired: 1 in, 7 out]
      n142 = call <vilib>:"Clear Errors.vi"("error in (no error)"=w322) -> ("error out"=w321:errorcluster)  [unwired: 1 in, 5 out]
    }
  }
  n143 = invoke class="VI" method="FP.Close"(error in=w9) -> (error out=w8:errorcluster)  [unwired: 2 in, 2 out]
  n144 = call <vilib>:"NI VeriStand - Signal When Ready for Shutdown.vi"("error in (no error)"=w8) -> ("error out"=→"error out":errorcluster)  [unwired: 10 out]
